vi "AddScale.vi"(8 "Gain (controlled by VSS)":dbl(slide)=1.0 caption="Gain" min=0.0 max=10.0 step=1.0 scale=0.0..10.0, 10 "Input 2":dbl, 11 "Input 1":dbl) -> (3 "Output":dbl)   [LabVIEW 2012]
panel:
  in  "Offset (controlled by LabVIEW)":dbl(slide) caption="Gain" min=0.0 max=10.0 step=1.0 scale=0.0..10.0
  # "Output = (Input1 + Input2) * Gain + Offset"
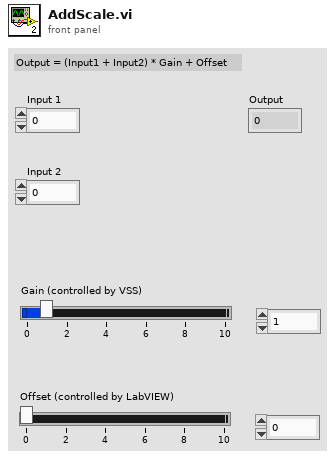
[diagram p1: front panel]
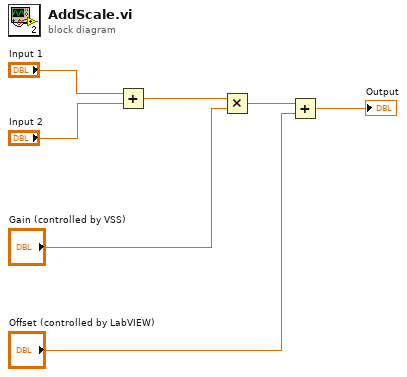
[diagram p0: block diagram]
diagram:
  n1 = Add(x="Input 1", y="Input 2") -> (x+y=w4:dbl)
  n2 = Multiply(x=w4, y="Gain (controlled by VSS)") -> (x*y=w3:dbl)
  n3 = Add(x=w3, y="Offset (controlled by LabVIEW)") -> (x+y=→"Output":dbl)
